vi "Wire Controls to When Call.vi"(8 "error in (no error)":errorcluster, 11 "VI in":refnum<vi>) -> (0 "error out":errorcluster, 3 "VI out":refnum<vi>)   [LabVIEW 2020, in "Mock Class Generator.lvclass"]
uses:
  Mock Class Generator.lvclass
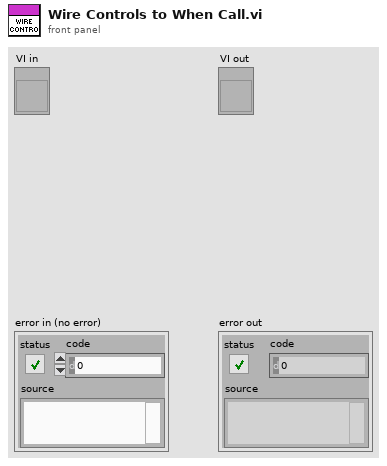
[diagram p1: front panel]
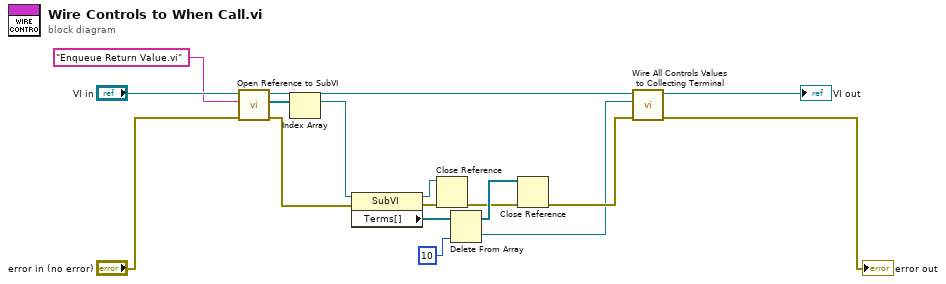
[diagram p0: block diagram]
diagram:
  n1 = call "Open Reference to SubVI.vi"("error in (no error)"="error in (no error)", "SubVI Name"="Enqueue Return Value.vi" ("y"), "VI in"="VI in") -> ("error out"=w6:errorcluster, "SubVIs"=w2:refnum<vi>[], "VI out"=w4:refnum<vi>)  [unwired: 6 in]
  n2 = Index Array(array=w2) -> (element=w1:refnum<vi>)  [unwired: 1 in]
  n3 = property class="SubVI"(reference=w1, error in=w6) -> (reference out=w13:refnum<vi>, error out=w12:errorcluster, "Terms[]"=w15:refnum<vi>[])
  n4 = Close Reference(reference=w13, error in (no error)=w12) -> (error out=w11:errorcluster)
  n5 = Delete From Array(array=w15, index=10) -> (deleted portion=w8:refnum<vi>, array with subset deleted=w14:refnum<vi>[])  [unwired: 1 in]
  n6 = Close Reference(reference=w14, error in (no error)=w11) -> (error out=w10:errorcluster)
  n7 = call "Wire All Controls Values to Collecting Terminal.vi"("error in (no error)"=w10, "Collecting Terminal"=w8, "VI in"=w4) -> ("error out"=→"error out":errorcluster, "VI out"=→"VI out":refnum<vi>)  [unwired: 7 in]
